vi "输出信息.vi"(1 "换行":bool, 2 "In":string, 3 "清空":bool) -> (0 "Out":string)   [LabVIEW 2011]
panel:
  out "换行符":string
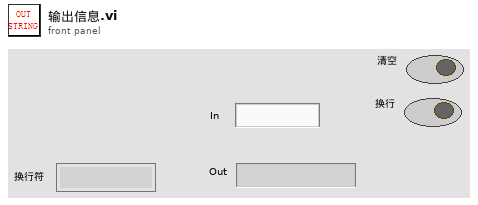
[diagram p1: front panel]
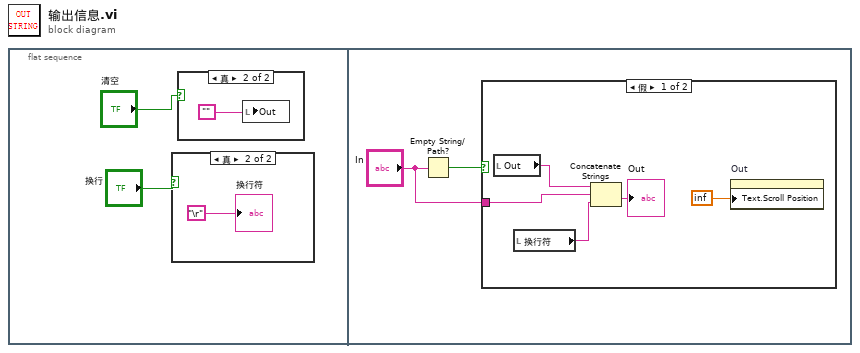
[diagram p0: block diagram]
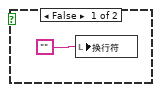
[diagram p3: hidden frame]
diagram:
  n1 = flat-sequence {
    frame #0 {
      n2 = case shown="真" "换行" {
        frame False {
          n3 = local write "换行符"("") -> ()
        }
        frame True {
          "换行符" <- "\r"
        }
      }
      n4 = case shown="真" "清空" {
        frame False {
        }
        frame True {
          n5 = local write "Out"("") -> ()
        }
      }
    }
    frame #1 {
      n6 = Empty String/Path?(string/path="In") -> (empty?=w6:bool)
      n7 = case shown="假" w6 {
        tunnel: "In" -> [w11 _]
        frame False {
          n8 = local read "Out"() -> (w10:string)
          n9 = local read "换行符"() -> (w9:string)
          n10 = Concatenate Strings(w10, w11, w9) -> (→"Out":string)
          n11 = property on="Out" class="Str"("Text.Scroll Position"=inf) -> ()  [unwired: 2 in, 2 out]
        }
        frame True {
        }
      }
    }
  }
